vi "To Test Event.vi"(11 "TestManagerMsg.Assertion in":refnum<class "TestManagerMsg.Assertion.lvclass">) -> (3 "Assert Event Data":T1={"name"="", "passed"=FALSE, "call-chain"=[], "test-error"={"status"=FALSE, "code"=0, "source"=""}, "timestamp"=timestamp(0 s since 1904-01-01), "assert-id"="", "test-id"="", "time"=-1.0, "message"="", "properties"=variant, "measurements"=variant, "user-defined"=variant})   [LabVIEW 2020, in "Caraya.lvlib" / "TestManagerMsg.Assertion.lvclass"]
uses:
  TestManagerMsg.Assertion.lvclass
  C:/projects/caraya/src/classes/Test Manager Message/TestManagerMsg.lvclass
  Test Result/Assert Event Data (Extended).ctl
  Test Manager Message/TestManagerMsg.lvclass/TestManagerMsg.ctl
  TestManagerMsg.Assertion.lvclass/TestManagerMsg.Assertion.ctl
  Test Manager Message/TestManagerMsg.lvclass
  Test Result/Test Result.lvclass
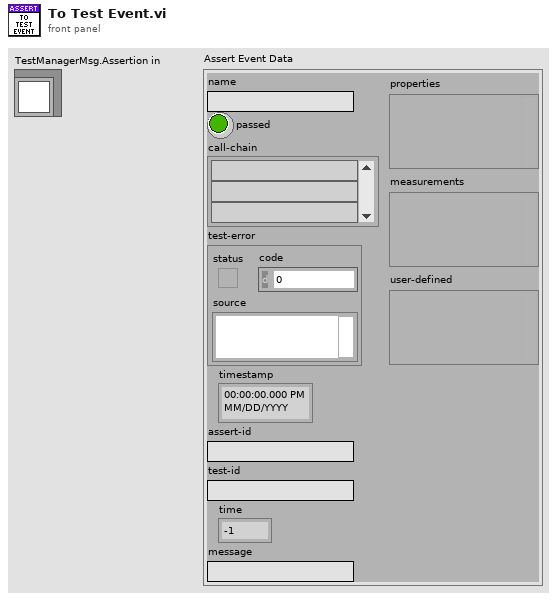
[diagram p1: front panel]
types:
  T1 = typedef "Caraya.lvlib/Test Result.lvclass/Assert Event Data (Extended).ctl" = cluster{"name":string, "passed":bool, "call-chain":string[], "test-error":errorcluster, "timestamp":timestamp, "assert-id":string, "test-id":string, "time":dbl, "message":string, "properties":variant, "measurements":variant, "user-defined":variant}
  T2 = typedef "Caraya.lvlib/TestManagerMsg.Assertion.lvclass/Assert-Data -- cluster.ctl" = cluster{"Label":string, "Asserted":bool, "call-chain":string[], "upstream-error":errorcluster, "timestamp":timestamp, "Execution time (s)":dbl}
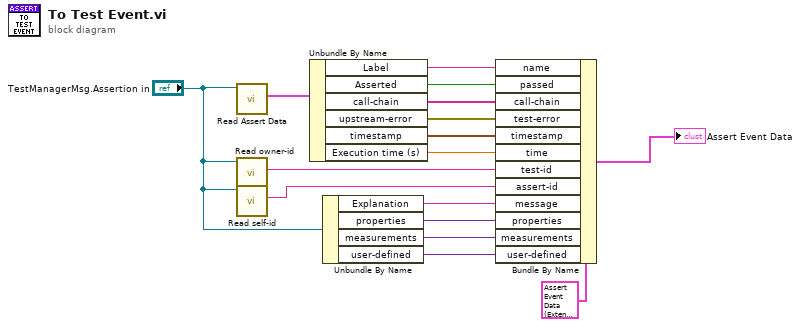
[diagram p0: block diagram]
diagram:
  n1 = call "Read Assert Data.vi"("Message Assertion"="TestManagerMsg.Assertion in") -> ("Assert Data"=w8:T2)  [unwired: 9 in, 1 out]
  n2 = call "Read owner-id.vi"("TestManagerMsg in"="TestManagerMsg.Assertion in") -> ("owner-id"=w15:string)  [unwired: 9 in, 1 out]
  n3 = call "Read self-id.vi"("TestManagerMsg in"="TestManagerMsg.Assertion in") -> ("self-id"=w16:string)  [unwired: 9 in, 1 out]
  n4 = Unbundle By Name(w8) -> ("Label"=w9:string, "Asserted"=w13:bool, "call-chain"=w12:string[], "upstream-error"=w11:errorcluster, "timestamp"=w10:timestamp, "Execution time (s)"=w14:dbl)
  n5 = Unbundle By Name("TestManagerMsg.Assertion in") -> ("Explanation"=w5:string, "properties"=w4:variant, "measurements"=w3:variant, "user-defined"=w2:variant)
  n6 = Bundle By Name(cluster=T1 {"name"="", "passed"=FALSE, "call-chain"=[], "test-error"={"status"=FALSE, "code"=0, "source"=""}, "timestamp"=timestamp(0 s since 1904-01-01), "assert-id"="", "test-id"="", "time"=-1.0, "message"="", "properties"=variant, "measurements"=variant, "user-defined"=variant} ("Assert Event Data"), "name"=w9, "passed"=w13, "call-chain"=w12, "test-error"=w11, "timestamp"=w10, "time"=w14, "test-id"=w15, "assert-id"=w16, "message"=w5, "properties"=w4, "measurements"=w3, "user-defined"=w2) -> (→"Assert Event Data":T1)
